vi "SPARK Configure Basic.vi"   [LabVIEW 2023]
doc: "Configure basic settings of the SPARK."
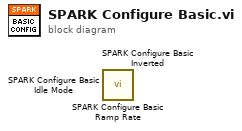
[diagram p0: block diagram]
diagram:
  n1 = call <vilib>:"SPARK Configure Basic Ramp Rate.vi"() -> ()  [unwired: 10 in, 2 out]
  n2 = call <vilib>:"SPARK Configure Basic Inverted.vi"() -> ()  [unwired: 10 in, 2 out]
  n3 = call <vilib>:"SPARK Configure Basic Idle Mode.vi"() -> ()  [unwired: 10 in, 2 out]
